vi "thermal_optical_capture_18.vi"() -> ()   [LabVIEW 2025]
uses:
  <vilib>/vision/driver/IMAQdx.llb/IMAQdx Acquisition Mode.ctl
  <vilib>/vision/driver/NI_Vision_Acquisition_Software.lvlib
panel:
  out "Optical Frame Out":string
  out "error out":errorcluster
  out "Times between Frames":u32
  out "Optical Preview":T1(plugin-control)
  in  "Camera Name":refnum<k21> caption="IMAQdx Session"
  in  "milliseconds to wait":u32=100
  out "Thermal Preview":T1(plugin-control)
  in  "Stop Preview":bool
  in  "STOP ACQUISITION":bool
  in  "Focus":dbl(slide) scale=0.0..100.0
  out "Thermal Frame Out":string
  in  "Output Folder":path
  in  "thermal capture interval (s)":dbl
  in  "Flag Button":bool
  in  "Stop & Save":bool
  in  "Record":bool
  # "Instructions:\n1) Make sure terminal is closed (from previous sessions)\n2) Inputs: Select camera, data folder path, & milliseconds to wait (~100)\n3) Run VI. (Optical images will begin writing, disregard.)\n4) Wait until terminal gives \"thermal camera calibrated and data reliable\" message\n5) Press Thermal Record \"Start\", both thermal & optical will write files with common timestamps"
  # "Thermal Record"
  # "(Enter \"28\")"
  # "^ append to base data folder \"...\\raw\\test_n\" for nth recording"
  # "(applies to thermal)"
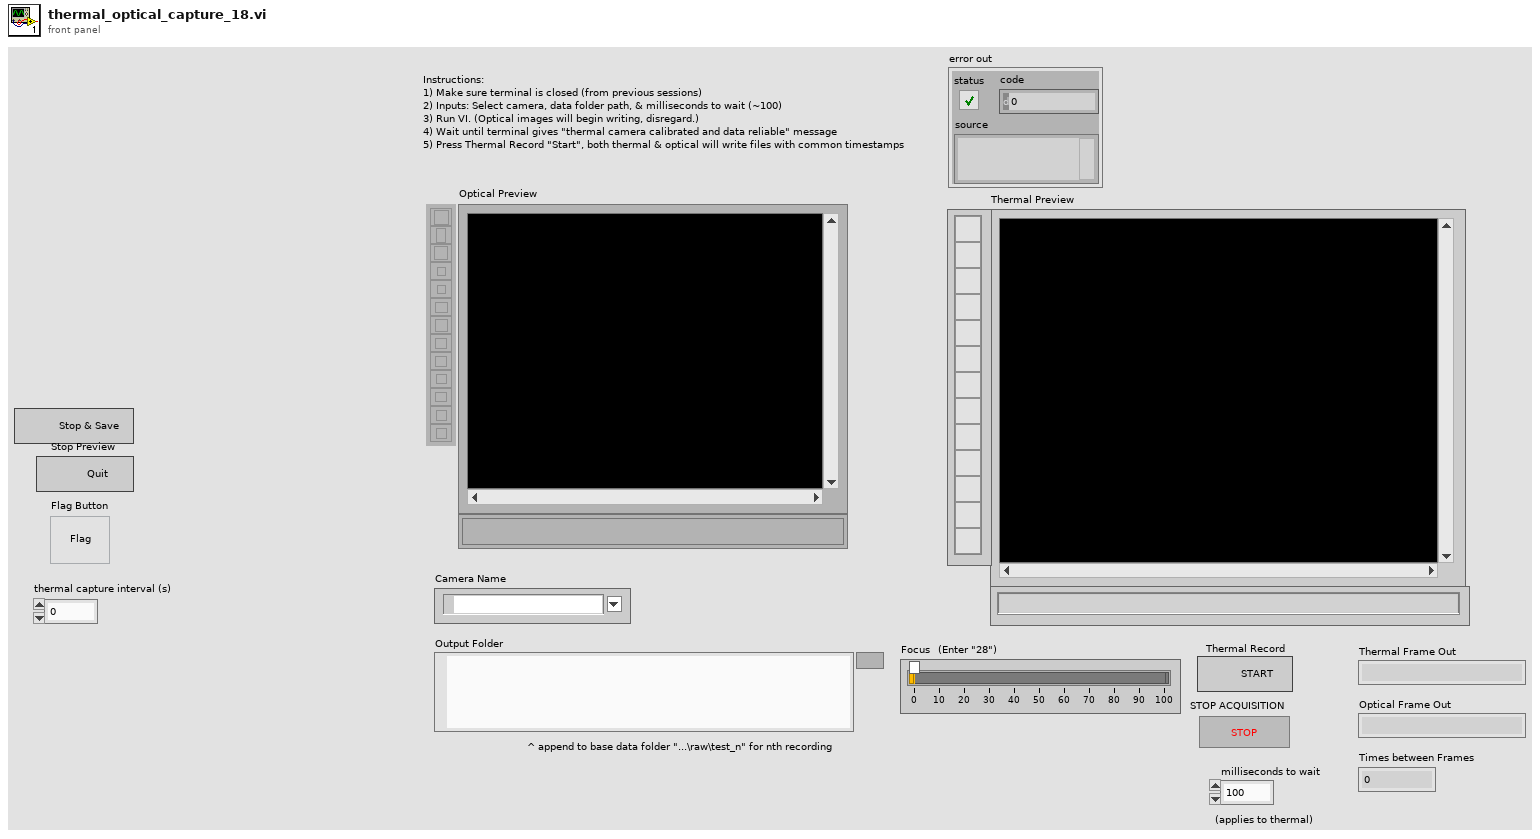
[diagram p1: front panel]
types:
  T1 = typedef "IMAQ Image.ctl" = refnum<image>
  T2 = typedef "NI_Vision_Acquisition_Software.lvlib/IMAQdx Acquisition Mode.ctl" = enum32{"One Shot", "Continuous"}
  T3 = enum16{"open", "replace", "create", "open or create", "replace or create", "replace or create with confirmation"}
  T4 = enum16{"big-endian, network order", "native, host order", "little-endian"}
  T5 = typedef "Image Type" = u32
  T6 = typedef "IMAQdx.ctl" = refnum<k21>
  T7 = enum16{"Standard", "Buffered", "CRLF", "Immediate"}
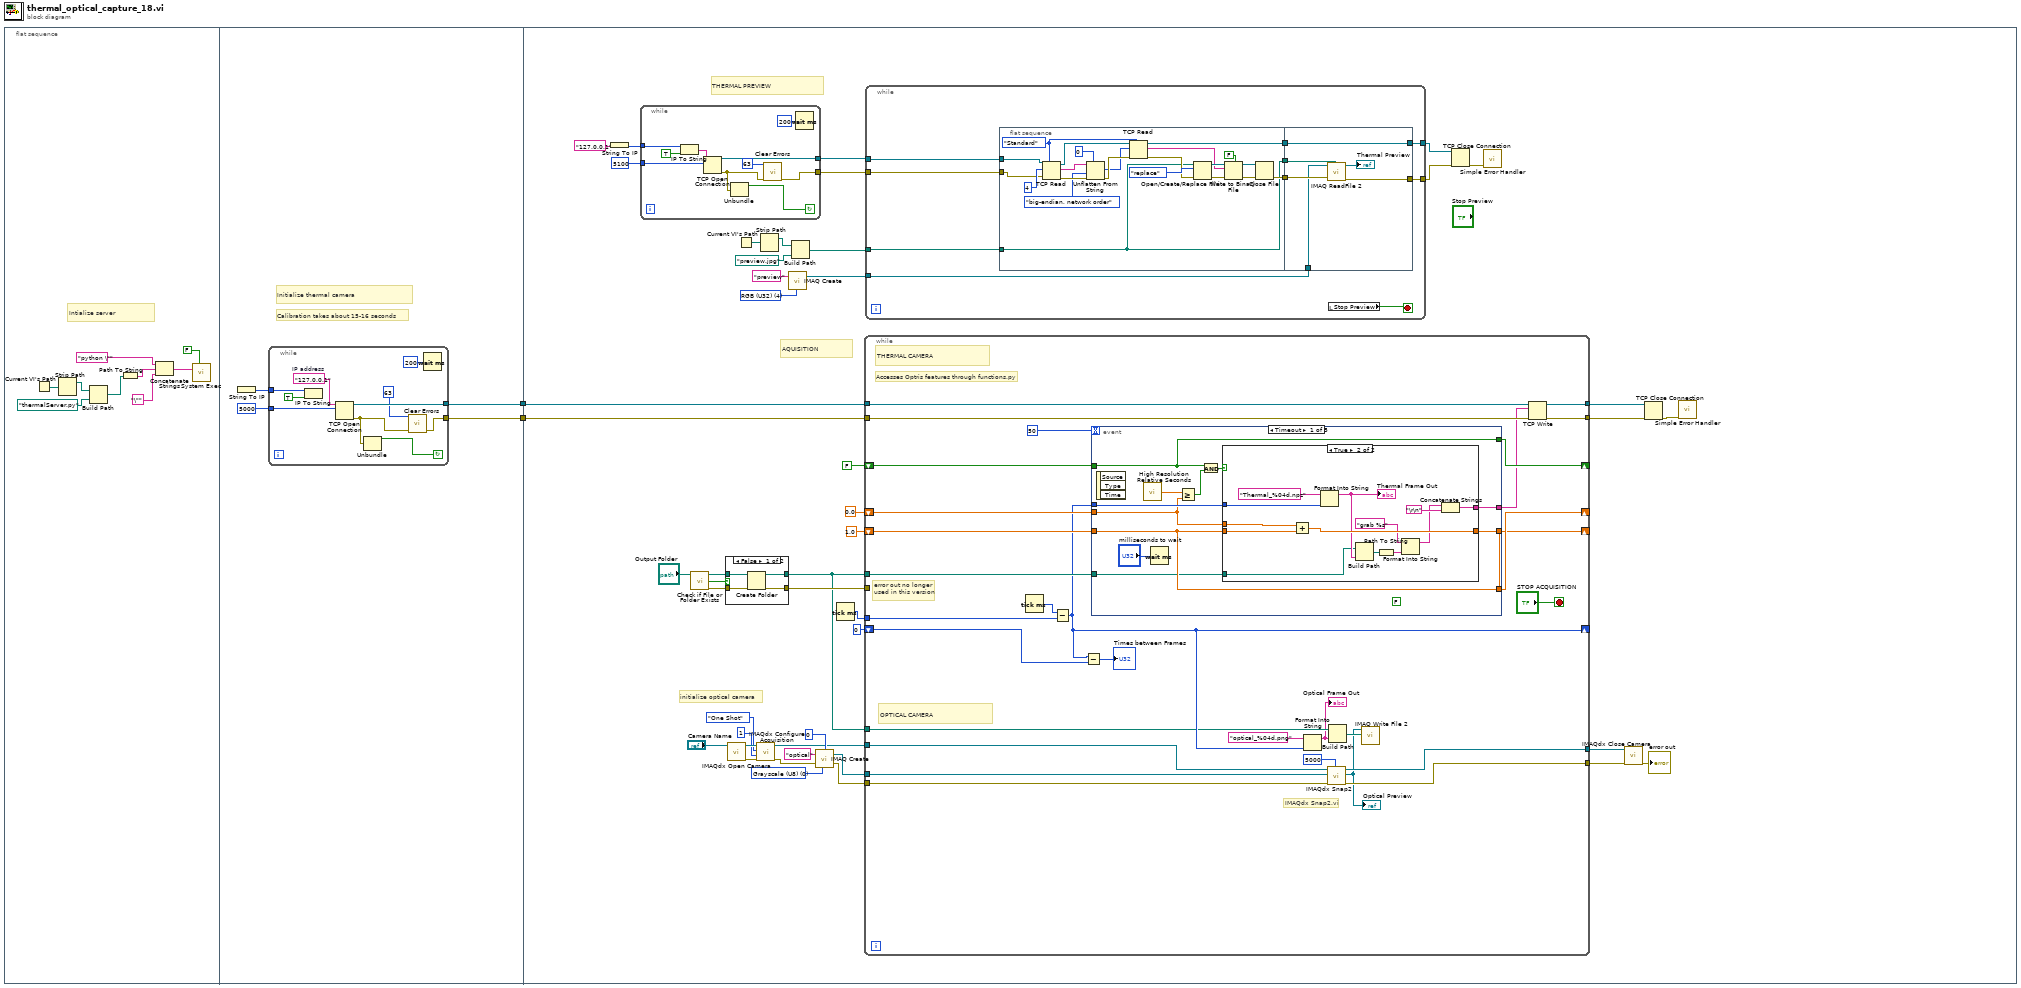
[diagram p0: block diagram]
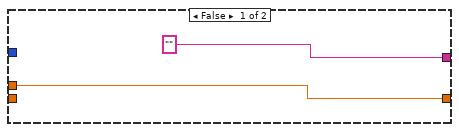
[diagram p3: hidden frame]
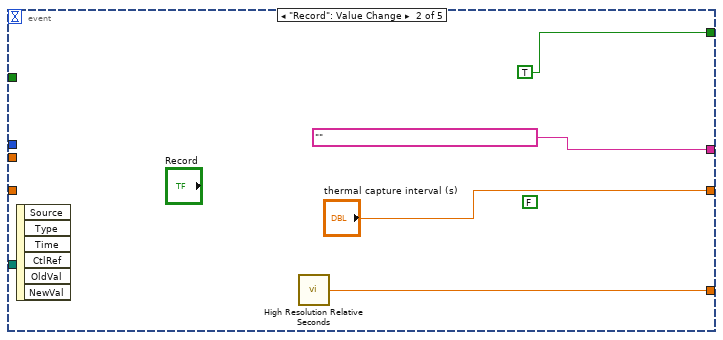
[diagram p4: hidden frame]
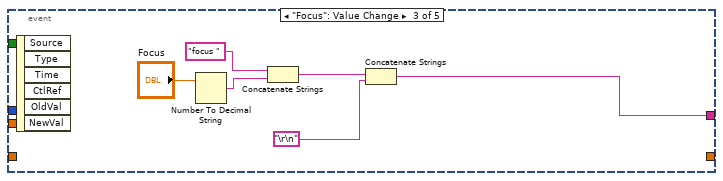
[diagram p5: hidden frame]
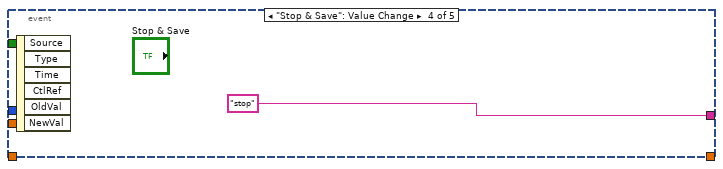
[diagram p6: hidden frame]
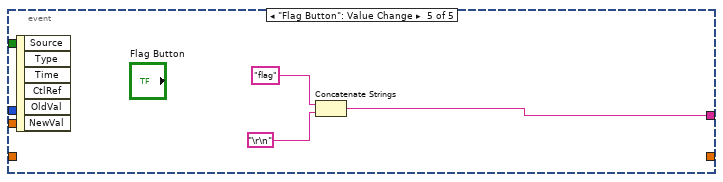
[diagram p7: hidden frame]
diagram:
  n1 = flat-sequence {
    tunnel: [w13] -> w2
    tunnel: [w12] -> w1
    tunnel: w1 -> [w67]
    tunnel: w2 -> [w66]
    frame #0 {
      # "Intialize server"
      n2 = Current VI's Path() -> (path=w6:path)
      n3 = Strip Path(path=w6) -> (stripped path=w7:path)  [unwired: 1 out]
      n4 = Build Path(base path=w7, name or relative path=path "thermalServer.py") -> (appended path=w4:path)
      n5 = Path To String(path=w4) -> (string=w10:string)
      n6 = Concatenate Strings("python \"" ("string"), w10, "\"" ("string")) -> (w9:string)
      n7 = call <vilib>:"System Exec.vi"("wait until completion? (T)"=FALSE, "command line"=w9) -> ()  [unwired: 6 in, 4 out]
    }
    frame #1 {
      # "Initialize thermal camera"
      # "Calibration takes about 15-16 seconds"
      n8 = String To IP() -> (0:w15:u32)  [unwired: 1 in]
      n9 = while {
        tunnel: [w20] -> w13
        tunnel: [w25] -> w12
        tunnel: w15 -> [w24]
        tunnel: u16 5000 ("remote port or service name") -> [w22]
        stop <- w17 continue-if-true
        w16 = "127.0.0.1"  # IP address
        n10 = IP To String(1:TRUE ("dot notation? (F)"), 2:w24) -> ()  [unwired: 1 out]
        n11 = TCP Open Connection(address=w16, remote port or service name=w22) -> (connection ID=w25:refnum<k5>, error out=w21:errorcluster)  [unwired: 3 in]
        n12 = Unbundle(w21) -> ("status"=w17:bool)  [unwired: 2 out]
        n13 = call <vilib>:"Clear Errors.vi"("error in (no error)"=w21, "specific error code to clear (0: all)"=63) -> ("error out"=w20:errorcluster)  [unwired: 4 in, 1 out]
        n14 = Wait (ms)(milliseconds to wait=u32 200) -> ()  [unwired: 1 out]
      }
    }
    frame #2 {
      w35 = T5 0 items=["Grayscale (U8)", "Grayscale (I16)", "Grayscale (SGL)", "Complex (CSG)", "RGB (U32)", "HSL (U32)", "RGB (U64)", "Grayscale (U16)"] ("Image Type")
      w55 = T5 4 items=["Grayscale (U8)", "Grayscale (I16)", "Grayscale (SGL)", "Complex (CSG)", "RGB (U32)", "HSL (U32)", "RGB (U64)", "Grayscale (U16)"] ("Image Type")
      # "initialize optical camera"
      # "THERMAL PREVIEW"
      # "AQUISITION"
      n15 = String To IP(1:"127.0.0.1" ("name")) -> (0:w54:u32)
      n16 = while {
        tunnel: w54 -> [w86]
        tunnel: [w80] -> w53
        tunnel: [w84] -> w52
        tunnel: u16 5100 ("remote port or service name") -> [w82]
        stop <- w77 continue-if-true
        n17 = IP To String(1:TRUE ("dot notation? (F)"), 2:w86) -> (0:w85:string)
        n18 = TCP Open Connection(address=w85, remote port or service name=w82) -> (connection ID=w84:refnum<k5>, error out=w81:errorcluster)  [unwired: 3 in]
        n19 = Unbundle(w81) -> ("status"=w77:bool)  [unwired: 2 out]
        n20 = call <vilib>:"Clear Errors.vi"("error in (no error)"=w81, "specific error code to clear (0: all)"=63) -> ("error out"=w80:errorcluster)  [unwired: 4 in, 1 out]
        n21 = Wait (ms)(milliseconds to wait=u32 200) -> ()  [unwired: 1 out]
      }
      n22 = call <vilib>:"Check if File or Folder Exists.vi"("path"="Output Folder") -> ("error out"=w47:errorcluster, "file or folder exists?"=w49:bool)  [unwired: 8 in, 1 out]
      n23 = case shown="False" w49 {
        tunnel: "Output Folder" -> [w74 w76]
        tunnel: [w73 w76] -> w29
        tunnel: w47 -> [w72 w75]
        tunnel: [w71 w75] -> w46
        frame False {
          n24 = Create Folder(path (use dialog)=w74, error in=w72) -> (created path=w73:path, error out=w71:errorcluster)  [unwired: 1 in, 1 out]
        }
        frame True {
        }
      }
      n25 = call <vilib>:"IMAQdx Open Camera.vi"("Session In"="Camera Name") -> ("error out"=w40:errorcluster, "Session Out"=w41:T6)  [unwired: 9 in]
      n26 = Current VI's Path() -> (path=w60:path)
      n27 = call <vilib>:"IMAQdx Configure Acquisition.vi"("error in"=w40, "Number of Buffers"=u32 1, "Continuous?"=IMAQdx_Acquisition_Mode."One Shot", "Session In"=w41) -> ("error out"=w38:errorcluster, "Session Out"=w30:T6)  [unwired: 6 in]
      n28 = Strip Path(path=w60) -> (stripped path=w61:path)  [unwired: 1 out]
      n29 = call "IMAQ Create"("Image Name"="preview", "Image Type"=w55) -> ("New Image"=w58:T1)  [unwired: 3 in, 1 out]
      n30 = Build Path(base path=w61, name or relative path=path "preview.jpg") -> (appended path=w59:path)
      n31 = call "IMAQ Create"("Border Size"=0, "Image Name"="optical", "Image Type"=w35, "error in (no error)"=w38) -> ("New Image"=w32:T1, "error out"=w31:errorcluster)  [unwired: 1 in]
      n32 = Tick Count (ms)() -> (millisecond timer value=w62:u32)
      n33 = while {
        tunnel: [w154] -> w68
        tunnel: [w153] -> w69
        tunnel: w67 -> [w152]
        tunnel: w66 -> [w151]
        shift-right: [w150] -> _
        shift-left: 0.0 -> [w147]
        shift-right: [w148] -> _
        shift-left: 1.0 -> [w145]
        shift-right: [w149] -> _
        shift-left: FALSE -> [w146]
        tunnel: w62 -> [w137]
        shift-right: [w136] -> _
        shift-left: u32 0 -> [w138]
        tunnel: w29 -> [w140]
        tunnel: w46 -> [_]
        tunnel: w32 -> [w135]
        tunnel: w31 -> [w134]
        tunnel: w30 -> [w133]
        tunnel: w29 -> [w132]
        tunnel: [w131] -> w27
        tunnel: [w130] -> w26
        stop <- "STOP ACQUISITION" stop-if-true
        # "IMAQdx Snap2.vi"
        # "OPTICAL CAMERA"
        # "error out no longer used in this version"
        # "THERMAL CAMERA"
        # "Accesses Optris features through functions.py"
        n34 = Tick Count (ms)() -> (millisecond timer value=w141:u32)
        n35 = Subtract(x=w141, y=w137) -> (x-y=w136:u32)
        n36 = Subtract(x=w136, y=w138) -> (x-y=→"Times between Frames":u32)
        n37 = event shown="[0] Timeout" {
          selector: _ -> [_ _ _ _ _]
          dyn-events: _ -> [_ _ _ _ _]
          timeout: 50 -> [_ _ _ _ _]
          tunnel: [w161 "" w185 "stop" w194] -> w142
          tunnel: w136 -> [w162 _ _ _ _]
          tunnel: [w159 w184 _ _ _] -> w150
          tunnel: [w157 TRUE _ _ _] -> w149
          tunnel: [w158 "thermal capture interval (s)" _ _ _] -> w148
          tunnel: w147 -> [w160 _ _ _ _]
          tunnel: w146 -> [w157 _ _ _ _]
          tunnel: w145 -> [w158 _ _ _ _]
          tunnel: w140 -> [w156 _ _ _ _]
          event Timeout {
            (unwired) FALSE
            n38 = event-data() -> ()  [unwired: 1 in, 3 out]
            n39 = call <vilib>:"High Resolution Relative Seconds.vi"() -> ("relative seconds"=w165:dbl)
            n40 = Wait (ms)(milliseconds to wait="milliseconds to wait") -> ()  [unwired: 1 out]
            n41 = Greater Or Equal?(x=w165, y=w160) -> (x >= y?=w164:bool)
            n42 = And(x=w157, y=w164) -> (x .and. y?=w163:bool)
            n43 = case shown="True" w163 {
              tunnel: w162 -> [_ w178]
              tunnel: ["" w179] -> w161
              tunnel: w160 -> [w166 w177]
              tunnel: w158 -> [_ w176]
              tunnel: [w166 w175] -> w159
              tunnel: w156 -> [_ w168]
              frame False {
              }
              frame True {
                n44 = Add(x=w177, y=w176) -> (x+y=w175:dbl)
                n45 = Format Into String(format string="Thermal_%04d.npz", w178) -> (resulting string=w169:string)  [unwired: 2 in, 1 out]
                "Thermal Frame Out" <- w169
                n46 = Build Path(base path=w168, name or relative path=w169) -> (appended path=w173:path)
                n47 = Path To String(path=w173) -> (string=w171:string)
                n48 = Format Into String(format string="grab %s", w171) -> (resulting string=w170:string)  [unwired: 2 in, 1 out]
                n49 = Concatenate Strings(w170, "\r\n") -> (w179:string)
              }
            }
          }
          event "Record": Value Change {
            (unwired) FALSE
            n50 = event-data() -> ()  [unwired: 1 in, 6 out]
            n51 = call <vilib>:"High Resolution Relative Seconds.vi"() -> ("relative seconds"=w184:dbl)
          }
          event "Focus": Value Change {
            n52 = event-data() -> ()  [unwired: 1 in, 6 out]
            n53 = Number To Decimal String(number="Focus") -> (decimal integer string=w190:string)  [unwired: 1 in]
            n54 = Concatenate Strings("focus ", w190) -> (w187:string)
            n55 = Concatenate Strings(w187, "\r\n") -> (w185:string)
          }
          event "Stop & Save": Value Change {
            n56 = event-data() -> ()  [unwired: 1 in, 6 out]
          }
          event "Flag Button": Value Change {
            n57 = event-data() -> ()  [unwired: 1 in, 6 out]
            n58 = Concatenate Strings("flag", "\r\n") -> (w194:string)
          }
        }
        n59 = Format Into String(format string="optical_%04d.png", w136) -> (resulting string=w125:string)  [unwired: 2 in, 1 out]
        "Optical Frame Out" <- w125
        n60 = call <vilib>:"IMAQdx Snap2.vi"("Timeout (ms)"=5000, "error in"=w134, "Image In"=w135, "Session In"=w133) -> ("error out"=w131:errorcluster, "Image Out"=w126:T1, "Session Out"=w130:T6)  [unwired: 5 in]
        "Optical Preview" <- w126
        n61 = Build Path(base path=w132, name or relative path=w125) -> (appended path=w128:path)
        n62 = call-poly "IMAQ Write File 2"("File Path"=w128, "Image"=w126) -> ()  [unwired: 8 in, 2 out]
        n63 = TCP Write(connection ID=w152, data in=w142, error in (no error)=w151) -> (connection ID out=w153:refnum<k5>, error out=w154:errorcluster)  [unwired: 1 in, 1 out]
      }
      n64 = while {
        tunnel: w58 -> [w91]
        tunnel: [w92] -> w44
        tunnel: [w96] -> w43
        tunnel: w59 -> [w94]
        tunnel: w53 -> [w89]
        tunnel: w52 -> [w88]
        stop <- w87 stop-if-true
        n65 = flat-sequence {
          tunnel: w94 -> [w100]
          tunnel: [w102] -> w95
          tunnel: [w101] -> w93
          tunnel: [w100] -> w90
          tunnel: w89 -> [w98]
          tunnel: w88 -> [w97]
          tunnel: [w124] -> w96
          tunnel: w95 -> [w124]
          tunnel: w93 -> [w123]
          tunnel: [w122] -> w92
          tunnel: w91 -> [w121]
          tunnel: w90 -> [w120]
          frame #0 {
            w111 = T7."Standard" ("mode (standard)")
            n66 = TCP Read(connection ID=w97, bytes to read=4, error in (no error)=w98, 7:w111) -> (connection ID out=w114:refnum<k5>, data out=w99:string, error out=w117:errorcluster)  [unwired: 1 in]
            n67 = Unflatten From String(type=0, binary string=w99, byte order (0:big-endian, network order)=T4."big-endian, network order", error in (no error)=w117) -> (value=w112:i32, error out=w113:errorcluster)  [unwired: 1 in, 1 out]
            n68 = TCP Read(connection ID=w114, bytes to read=w112, error in (no error)=w113, 7:w111) -> (connection ID out=w102:refnum<k5>, data out=w107:string, error out=w109:errorcluster)  [unwired: 1 in]
            n69 = Open/Create/Replace File(file path (use dialog)=w100, error in=w109, operation (0:open)=T3."replace") -> (refnum out=w108:refnum<file>, error out=w105:errorcluster)  [unwired: 3 in, 1 out]
            n70 = Write to Binary File(file (use dialog)=w108, data=w107, error in=w105, 5:FALSE ("prepend array or string size? (T)")) -> (refnum out=w103:refnum<file>, error out=w104:errorcluster)  [unwired: 2 in, 1 out]
            n71 = Close File(refnum=w103, error in=w104) -> (error out=w101:errorcluster)  [unwired: 1 out]
          }
          frame #1 {
            n72 = call "IMAQ ReadFile 2"("File Path"=w120, "error in (no error)"=w123, "Image"=w121) -> ("error out"=w122:errorcluster, "Image Out"=→"Thermal Preview":T1)  [unwired: 4 in, 3 out]
          }
        }
        n73 = local read "Stop Preview"() -> (w87:bool)
      }
      n74 = TCP Close Connection(connection ID=w43, error in (no error)=w44) -> (error out=w45:errorcluster)  [unwired: 1 in, 1 out]
      n75 = call <vilib>:"Simple Error Handler.vi"("error in (no error)"=w45) -> ()  [unwired: 4 in, 5 out]
      n76 = call <vilib>:"IMAQdx Close Camera.vi"("error in"=w27, "Session In"=w26) -> ("error out"=→"error out":errorcluster)  [unwired: 9 in]
      n77 = TCP Close Connection(connection ID=w69, error in (no error)=w68) -> (error out=w70:errorcluster)  [unwired: 1 in, 1 out]
      n78 = call <vilib>:"Simple Error Handler.vi"("error in (no error)"=w70) -> ()  [unwired: 4 in, 5 out]
    }
  }
